vi "libssh2_knownhost_addc.vi"(4 "comment":string, 6 "salt":string, 7 "typemask":T2 items=["TYPE_PLAIN"=1, "TYPE_SHA1"=2, "TYPE_CUSTOM"=3, "KEYENC_RAW"=65536, "KEYENC_BASE64"=131072, "KEY_RSA1"=262144, "KEY_SSHRSA"=524288, "KEY_SSHDSS (deprecated)"=786432, "KEY_ECDSA_256"=1048576, "KEY_ECDSA_384"=1310720, "KEY_ECDSA_521"=1572864, "KEY_ED25519"=1835008, "KEY_UNKNOWN"=3932160], 8 "error in (no error)":errorcluster, 9 "key":u8[](array[numeric]), 10 "hostname":string, 11 "host key database":T3) -> (0 "error out":errorcluster, 3 "host key":T1)   [LabVIEW 2017, in "libssh2.lvlib"]
doc: "Add a host key to a host key database."
uses:
  libssh2.lvlib
  Host Key Database Refnum.ctl
  libssh2_knownhost_typemask.ctl
  Host Key Refnum.ctl
  Warn Deprecated.vi
  Not A Host Key Database.vi
  <vilib>/Utility/error.llb/Error Cluster From Error Code.vi
  Global Settings.vi
  Read Host Key Database Refnum.vi
  <vilib>/Utility/semaphor.llb/Acquire Semaphore.vi
  <vilib>/Utility/semaphor.llb/Release Semaphore.vi
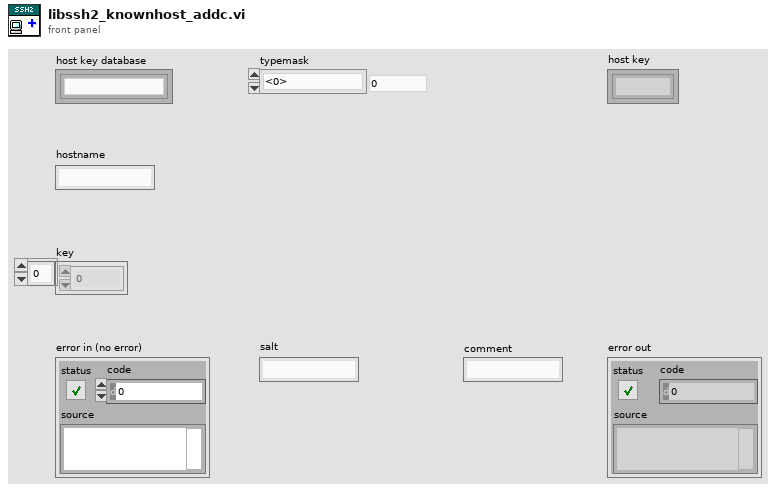
[diagram p1: front panel]
types:
  T1 = typedef "libssh2.lvlib/Host Key Refnum.ctl" = refnum<k1>
  T2 = typedef "libssh2.lvlib/libssh2_knownhost_typemask.ctl" = i32
  T3 = typedef "libssh2.lvlib/Host Key Database Refnum.ctl" = refnum<k1>
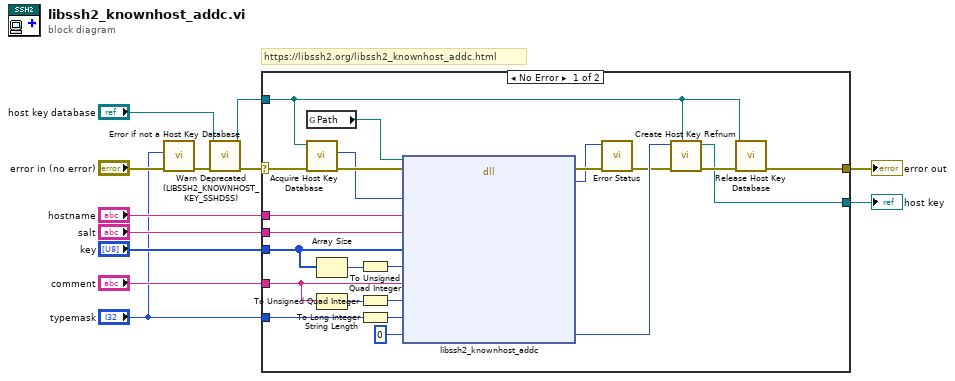
[diagram p0: block diagram]
diagram:
  # "https://libssh2.org/libssh2_knownhost_addc.html"
  n1 = call "Warn Deprecated (LIBSSH2_KNOWNHOST_KEY_SSHDSS).vi"("error in (no error)"="error in (no error)", "typemask"="typemask") -> ("error out"=w2:errorcluster)  [unwired: 9 in]
  n2 = call "Error if not a Host Key Database.vi"("error in (no error)"=w2, "host key database"="host key database") -> ("error out"=w11:errorcluster, "host key database out"=w9:T3)  [unwired: 8 in]
  n3 = case shown="No Error" w11 {
    selector: w11 -> [w13 w36]
    tunnel: [w16 w36] -> w12
    tunnel: w9 -> [w15 _]
    tunnel: [w34 _] -> w8
    tunnel: "typemask" -> [w14 _]
    tunnel: "comment" -> [w20 _]
    tunnel: "key" -> [w22 _]
    tunnel: "salt" -> [w25 _]
    tunnel: "hostname" -> [w24 _]
    frame No Error {
      n4 = global read "Global Settings.vi" "Path"() -> (w29:path)
      n5 = call "Acquire Host Key Database.vi"("error in (no error)"=w13, "host key database"=w15) -> ("error out"=w32:errorcluster, "LIBSSH2_KNOWNHOSTS*"=w31:u64)  [unwired: 8 in]
      n6 = Array Size(array=w22) -> (size(s)=w23:i32)
      n7 = String Length(string=w20) -> (length=w21:i32)
      n8 = To Unsigned Quad Integer(1:w23) -> (0:w19:u64)
      n9 = To Unsigned Quad Integer(1:w21) -> (0:w18:u64)
      n10 = To Long Integer(number=w14) -> (32bit integer=w17:T2)
      n11 = dll-call lib="?" fn="libssh2_knownhost_addc"(path in=w29, error in=w32, "hosts"=w31, "host"=w24, "salt"=w25, "key"=w22, "keylen"=w19, "comment"=w20, "commentlen"=w18, "typemask"=w17, "store"=u64 0) -> (error out=w33:errorcluster, "return value"=w27:i32, "store"=w30:u64)  [unwired: 9 in, 1 out]
      n12 = call "Error Status.vi"("error in (no error)"=w33, "return value"=w27) -> ("error out"=w28:errorcluster)  [unwired: 8 in, 1 out]
      n13 = call "Create Host Key Refnum.vi"("host key database"=w15, "error in (no error)"=w28, "libssh2_knownhost*"=w30) -> ("error out"=w35:errorcluster, "host key"=w34:T1)  [unwired: 7 in]
      n14 = call "Release Host Key Database.vi"("error in (no error)"=w35, "host key database"=w15) -> ("error out"=w16:errorcluster)  [unwired: 9 in]
    }
    frame Error {
    }
  }
  "error out" <- w12
  "host key" <- w8
